vi "List Drivers.vi"(11 "error in (no error)":errorcluster) -> (15 "error out":errorcluster)   [LabVIEW 2021, in "Migrator.lvlib"]
uses:
  Migrator.lvlib
  <vilib>/Utility/traverseref.llb/TRef TravTarget.ctl
  <vilib>/Utility/traverseref.llb/VI Scripting - Traverse.lvlib
  Migrator Reusables/Migrator Reusables.lvlib
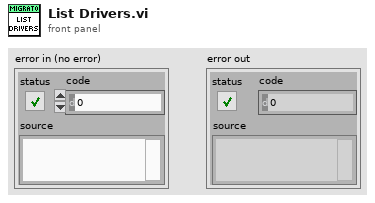
[diagram p1: front panel]
types:
  T1 = typedef "TRef TravTarget.ctl" = enum16{"FP", "BD", "Other"}
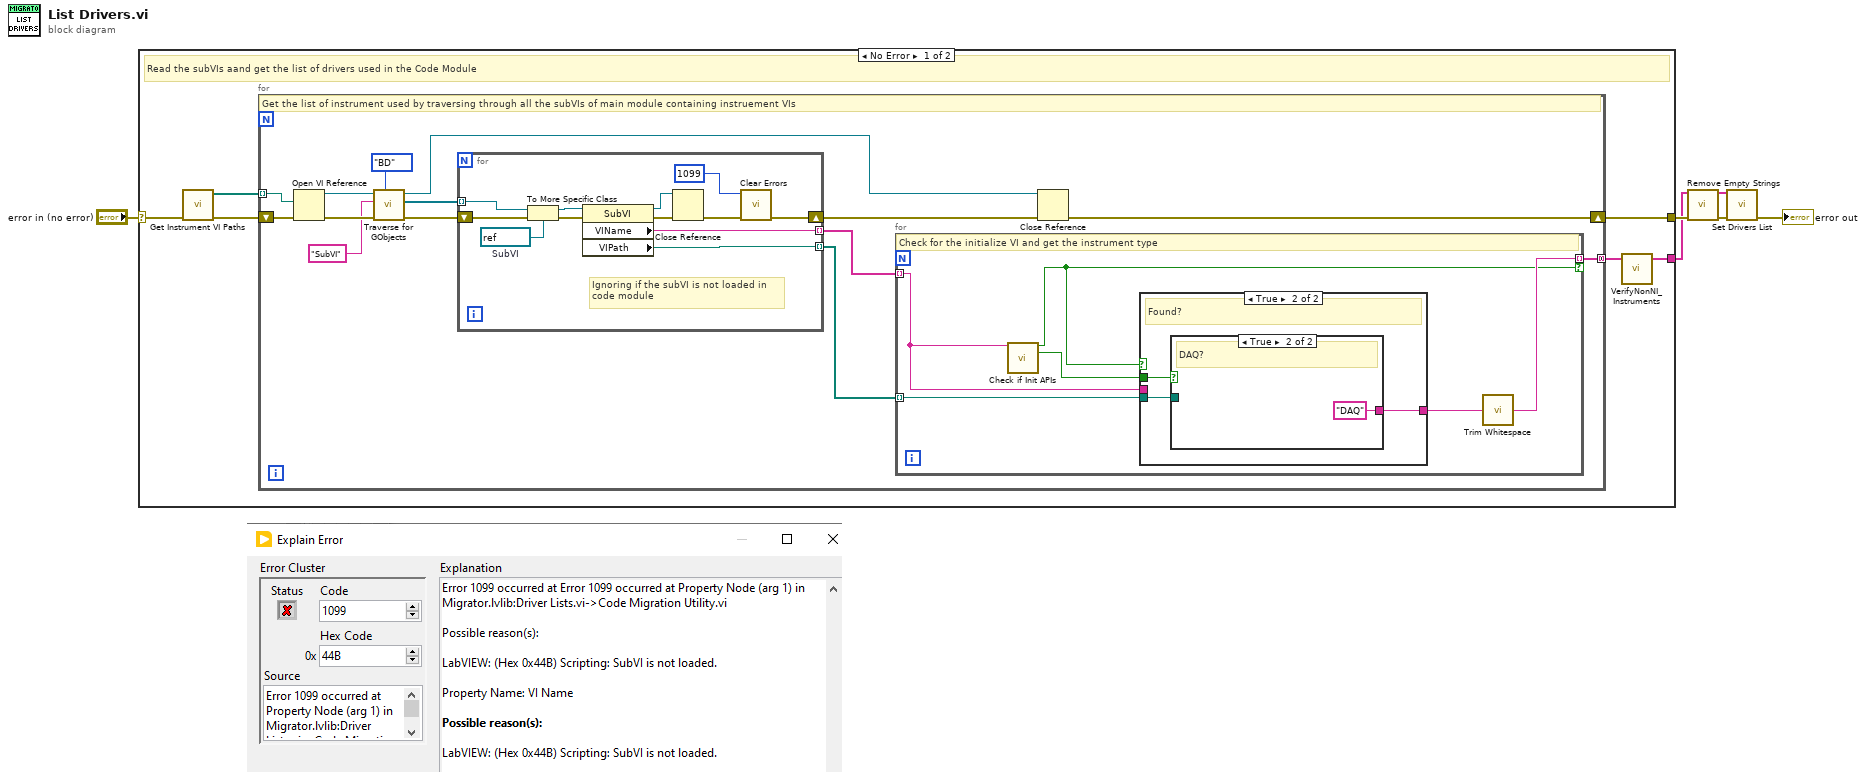
[diagram p0: block diagram]
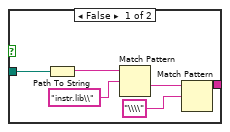
[diagram p3: hidden frame]
diagram:
  n1 = case shown="No Error" "error in (no error)" {
    selector: "error in (no error)" -> [w10 w54]
    tunnel: [w6 w54] -> w4
    tunnel: [w7 _] -> w2
    frame No Error {
      # "Read the subVIs aand get the list of drivers used in the Code Module"
      n2 = call "Get Instrument VI Paths.vi"("error in (no error)"=w10) -> ("error out"=w9:errorcluster, "Instr VI Paths[]"=w11:path[])  [unwired: 9 in]
      n3 = for {
        tunnel: w11 -> [w20] mode=indexing
        tunnel: [w16] -> w8 mode=concatenating
        shift-right: [w14] -> w6
        shift-left: w9 -> [w19]
        # "Get the list of instrument used by traversing through all the subVIs of main module containing instruement VIs"
        n4 = Open VI Reference(vi path=w20, error in (no error)=w19) -> (vi reference=w15:refnum<vi>, error out=w23:errorcluster)  [unwired: 4 in]
        n5 = call <vilib>:"Traverse for GObjects.vi"("Traverse Target"=TRef_TravTarget."BD", "error in (no error)"=w23, "Class Name"="SubVI", "VI Refnum"=w15) -> ("error out"=w25:errorcluster, "References"=w24:refnum<vi>[], "dup VI Refnum"=w12:refnum<vi>)  [unwired: 4 in, 1 out]
        n6 = for {
          tunnel: w24 -> [w52] mode=indexing
          tunnel: [w48] -> w18 mode=indexing
          tunnel: [w47] -> w17 mode=indexing
          shift-right: [w43] -> w13
          shift-left: w25 -> [w51]
          w53 = refnum<vi> refnum  # SubVI
          # "Ignoring if the subVI is not loaded in\ncode module"
          n7 = To More Specific Class(target class=w53, reference=w52, error in=w51) -> (specific class reference=w50:refnum<vi>, error out=w49:errorcluster)
          n8 = property class="SubVI"(reference=w50, error in=w49) -> (reference out=w46:refnum<vi>, error out=w45:errorcluster, "VIName"=w48:string, "VIPath"=w47:path)
          n9 = Close Reference(reference=w46, error in (no error)=w45) -> (error out=w44:errorcluster)
          n10 = call <vilib>:"Clear Errors.vi"("error in (no error)"=w44, "specific error code to clear (0: all)"=1099) -> ("error out"=w43:errorcluster)  [unwired: 4 in, 1 out]
        }
        n11 = for {
          tunnel: w18 -> [w27] mode=indexing
          tunnel: w17 -> [w31] mode=indexing
          tunnel: [w30] -> w16 mode=indexing if=w28
          # "Check for the initialize VI and get the instrument type"
          n12 = call "Check if Init APIs.vi"("VIName"=w27) -> ("Instrument Driver Found?"=w28:bool, "DAQ?"=w26:bool)  [unwired: 13 in]
          n13 = case shown="True" w28 {
            tunnel: w31 -> [_ w34]
            tunnel: [_ w33] -> w29
            tunnel: w27 -> [_ _]
            tunnel: w26 -> [_ w32]
            frame False {
            }
            frame True {
              # "Found?"
              n14 = case shown="True" w32 {
                tunnel: w34 -> [w36 _]
                tunnel: [w35 "DAQ"] -> w33
                frame False {
                  n15 = Path To String(path=w36) -> (string=w37:string)
                  n16 = Match Pattern(string=w37, regular expression="instr.lib\\") -> (after substring=w39:string)  [unwired: 1 in, 3 out]
                  n17 = Match Pattern(string=w39, regular expression="\\\\") -> (before substring=w35:string)  [unwired: 1 in, 3 out]
                }
                frame True {
                  # "DAQ?"
                }
              }
            }
          }
          n18 = call <vilib>:"Trim Whitespace.vi"("string"=w29) -> ("trimmed string"=w30:string)  [unwired: 1 in]
        }
        n19 = Close Reference(reference=w12, error in (no error)=w13) -> (error out=w14:errorcluster)
      }
      n20 = call "VerifyNonNI_Instruments.vi"("Instrument Types In"=w8) -> ("Instrument Types Out"=w7:string[])  [unwired: 4 in]
    }
    frame Error {
    }
  }
  n21 = call "Remove Empty Strings.vi"("Instrument Types Out in"=w2) -> ("Instrument Types Out out"=w1:string[])  [unwired: 14 in]
  n22 = call "Set Drivers List.vi"("Name"=w1, "error in (no error)"=w4) -> ("error out"=→"error out":errorcluster)  [unwired: 13 in]
